vi "VIH Utility - UI - Make Row Visible (MC Listbox).vi"(8 "error in":errorcluster, 10 "Row":i32, 11 "MC Listbox Refnum":refnum<vi>) -> (0 "error out":errorcluster, 3 "dup MC Listbox Refnum":refnum<vi>)   [LabVIEW 2014]
doc: "::: VI Helpeks :::\nCopyright (c) 2000-2026 Konstantin Shifershteyn. All rights reserved."
uses:
  <vilib>/Utility/miscctls.llb/LVRowAndColumnUnsignedTypeDef.ctl
panel:
  # "VI Helpeks\nCopyright (c) 2012-2026 Konstantin Shifershteyn"
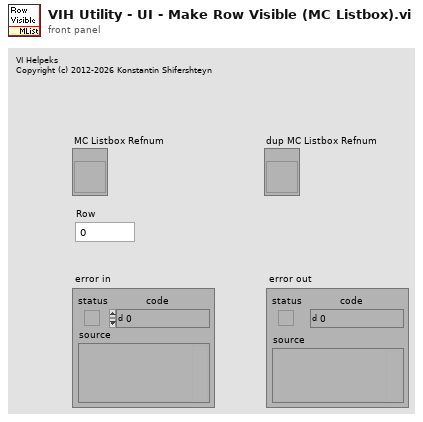
[diagram p1: front panel]
types:
  T1 = typedef "LVRowAndColumnUnsignedTypeDef.ctl" = cluster{"Row":u32, "Column":u32}
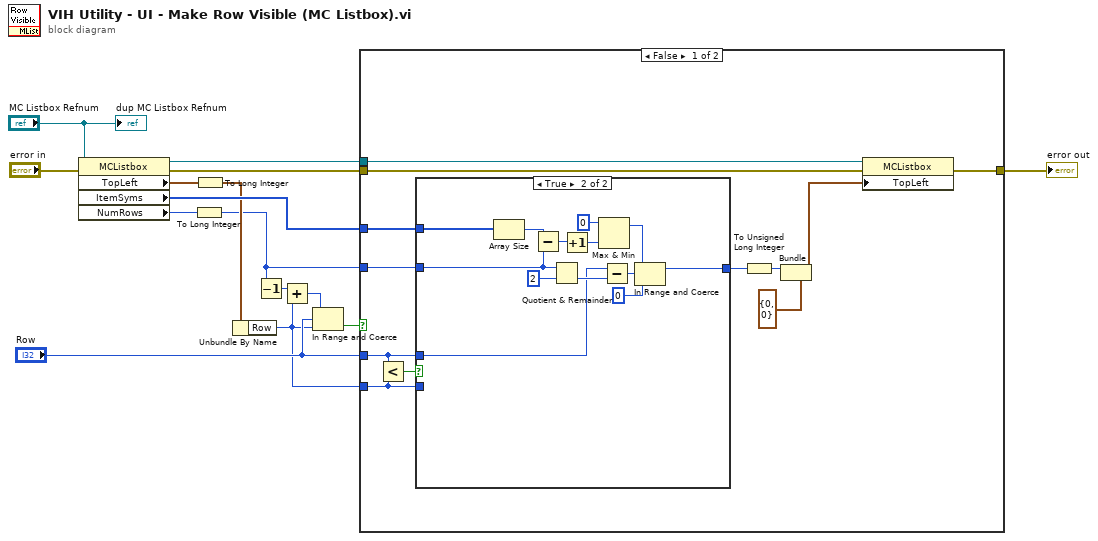
[diagram p0: block diagram]
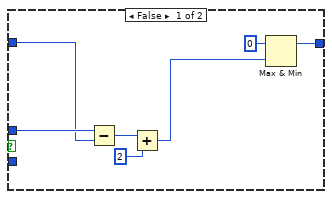
[diagram p2: hidden frame]
diagram:
  n1 = property on="Property Node" class="MCListbox"(reference="MC Listbox Refnum", error in="error in") -> (reference out=w14:refnum<vi>, error out=w12:errorcluster, "TopLeft"=w9:T1, "ItemSyms"=w15:i32[], "NumRows"=w7:u32)
  n2 = To Long Integer(number=w7) -> (32bit integer=w3:i32)
  n3 = To Long Integer(number=w9) -> (32bit integer=w5:cluster{"Row":i32, "Column":i32})
  n4 = Unbundle By Name(w5) -> ("Row"=w1:i32)
  n5 = Decrement(x=w3) -> (x-1=w8:i32)
  n6 = Add(x=w8, y=w1) -> (x+y=w6:i32)
  n7 = In Range and Coerce(upper limit=w6, x="Row", lower limit=w1) -> (In Range?=w2:bool)  [unwired: 1 out]
  n8 = case shown="False" w2 {
    tunnel: w15 -> [w23 _]
    tunnel: w14 -> [w22 _]
    tunnel: w12 -> [w21 w48]
    tunnel: [w20 w48] -> w10
    tunnel: "Row" -> [w18 _]
    tunnel: w3 -> [w19 _]
    tunnel: w1 -> [w16 _]
    frame False {
      n9 = Less?(x=w18, y=w16) -> (x < y?=w17:bool)
      n10 = case shown="True" w17 {
        tunnel: [w33 w46] -> w27
        tunnel: w23 -> [_ w37]
        tunnel: w19 -> [w30 w36]
        tunnel: w18 -> [w34 w35]
        tunnel: w16 -> [_ _]
        frame False {
          n11 = Subtract(x=w34, y=w30) -> (x-y=w29:i32)
          n12 = Add(x=w29, y=2) -> (x+y=w31:i32)
          n13 = Max & Min(x=0, y=w31) -> (max(x,y)=w33:i32)  [unwired: 1 out]
        }
        frame True {
          n14 = Array Size(array=w37) -> (size(s)=w42:i32)
          n15 = Subtract(x=w42, y=w36) -> (x-y=w43:i32)
          n16 = Quotient & Remainder(x=w36, y=2) -> (floor(x/y)=w39:i32)  [unwired: 1 out]
          n17 = Increment(x=w43) -> (x+1=w44:i32)
          n18 = Max & Min(x=0, y=w44) -> (max(x,y)=w47:i32)  [unwired: 1 out]
          n19 = Subtract(x=w35, y=w39) -> (x-y=w40:i32)
          n20 = In Range and Coerce(upper limit=w47, x=w40, lower limit=0 ("x")) -> (coerced(x)=w46:i32)  [unwired: 1 out]
        }
      }
      n21 = To Unsigned Long Integer(number=w27) -> (unsigned 32bit integer=w26:u32)
      n22 = Bundle(cluster=T1 {"Row"=0, "Column"=0} ("Top Left Visible Cell"), "Row"=w26) -> (w25:T1)  [unwired: 1 in]
      n23 = property on="Property Node" class="MCListbox"(reference=w22, error in=w21, "TopLeft"=w25) -> (error out=w20:errorcluster)  [unwired: 1 out]
    }
    frame True {
    }
  }
  "error out" <- w10
  "dup MC Listbox Refnum" <- "MC Listbox Refnum"
